vi "Set Legend (WFGraph).vi"(8 "error in (no error)":errorcluster, 10 "Plot.Plot Name":string[](array[string]), 11 "WFGraph in":refnum<vi>) -> (0 "error out":errorcluster)   [LabVIEW 2019, in "Instrument.Lockin.lvlib" / "Instrument UI.Lockin.lvclass"]
uses:
  Instrument UI.Lockin.lvclass
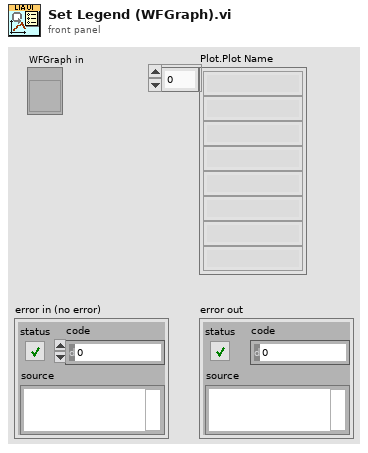
[diagram p1: front panel]
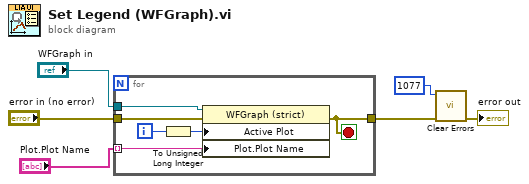
[diagram p0: block diagram]
diagram:
  n1 = for {
    tunnel: "Plot.Plot Name" -> [w10] mode=indexing
    tunnel: "WFGraph in" -> [w8]
    tunnel: "error in (no error)" -> [w12]
    tunnel: [w7] -> w5
    i -> [w9]
    stop <- w7 stop-if-true
    n2 = To Unsigned Long Integer(number=w9) -> (unsigned 32bit integer=w11:u32)
    n3 = property on="Property Node" class="WFGraph (strict)"(reference=w8, error in=w12, "Active Plot"=w11, "Plot.Plot Name"=w10) -> (error out=w7:errorcluster)  [unwired: 1 out]
  }
  n4 = call <vilib>:"Clear Errors.vi"("error in (no error)"=w5, "specific error code to clear (0: all)"=1077) -> ("error out"=→"error out":errorcluster)  [unwired: 4 in, 1 out]
